vi "from string.vi"(8 "error in":errorcluster, 9 "data":string, 10 "version":string, 11 "Modbus Slave configuration in":refnum<class "Modbus Module configuration.lvclass">) -> (0 "error out":errorcluster, 3 "Modbus Slave configuration out":refnum<class "Modbus Module configuration.lvclass">)   [LabVIEW 2015, in "Modbus Module configuration.lvclass"]
doc: "Provides an interface for loading a module configuration from a file or other serialized data source. It is recommended that all children of this class store data in two sets--data required for its own initialization, and any data required for parent initialization--and that each implementation uses the <b>Call Parent Method</b> primitive to de-serialize parent information. As a result, it is expected that every module configuration class calls <b>component configuration.lvclass:From String.vi</b>.Platypus Framework 1.0.1.65\nNI Systems Engineering - National Instruments"
uses:
  Modbus Module configuration.lvclass
  module channel/Modbus Module Channel.lvclass
  modbus class.ctl
  Modbus Module configuration.lvclass/Modbus Module configuration.ctl
  <vilib>/NI/Tag Bus Module Framework/module configuration/TBM module configuration.lvclass
  <vilib>/NI/Configuration Framework/serializable configuration/NISE_CEF_serializable configuration.lvclass
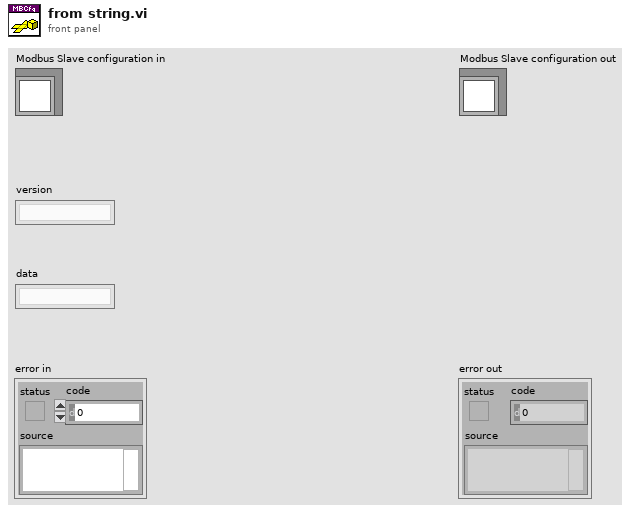
[diagram p1: front panel]
types:
  T1 = typedef "Modbus Module configuration.lvclass/modbus class.ctl" = enum16{"TCP master", "TCP slave", "serial master", "serial slave"}
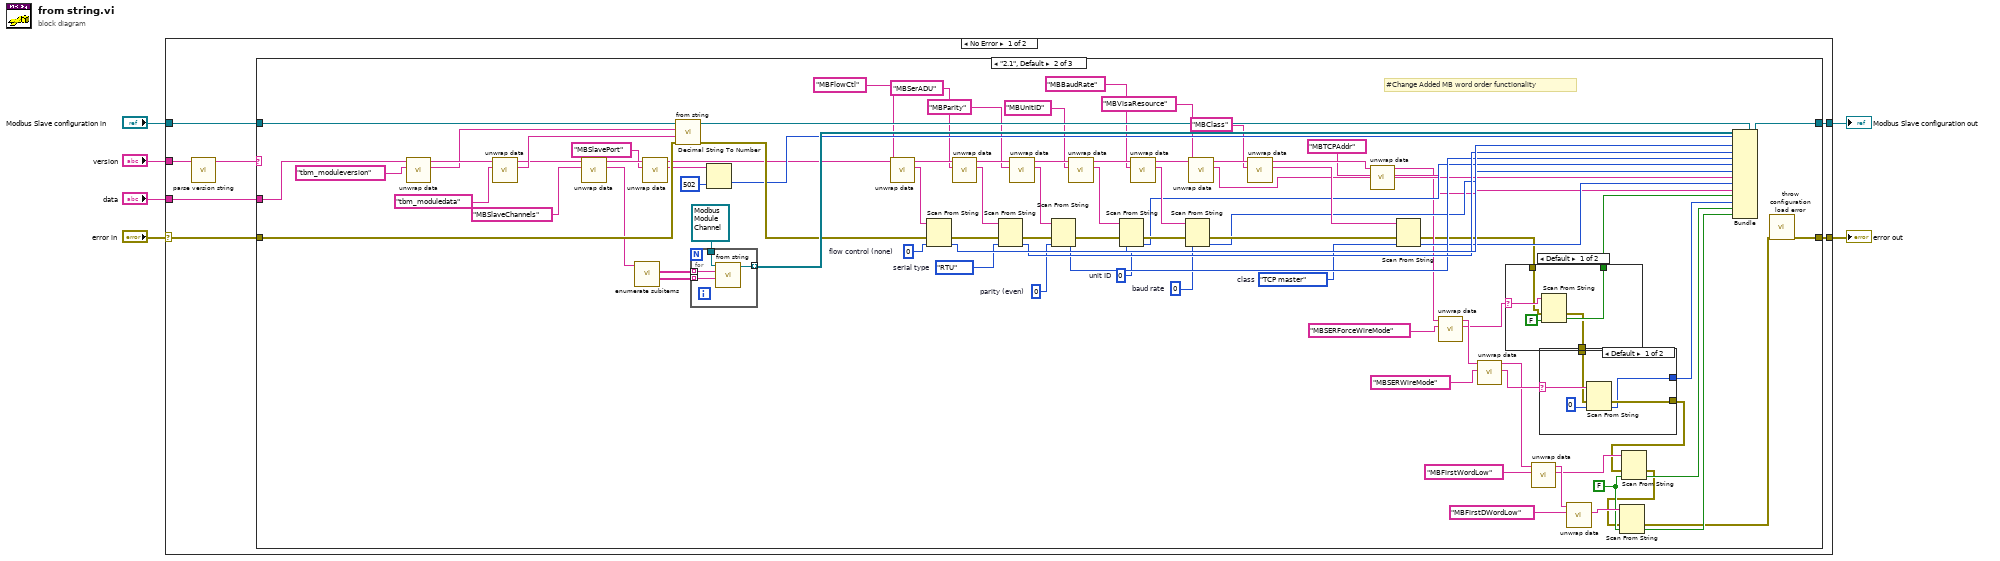
[diagram p0: block diagram]
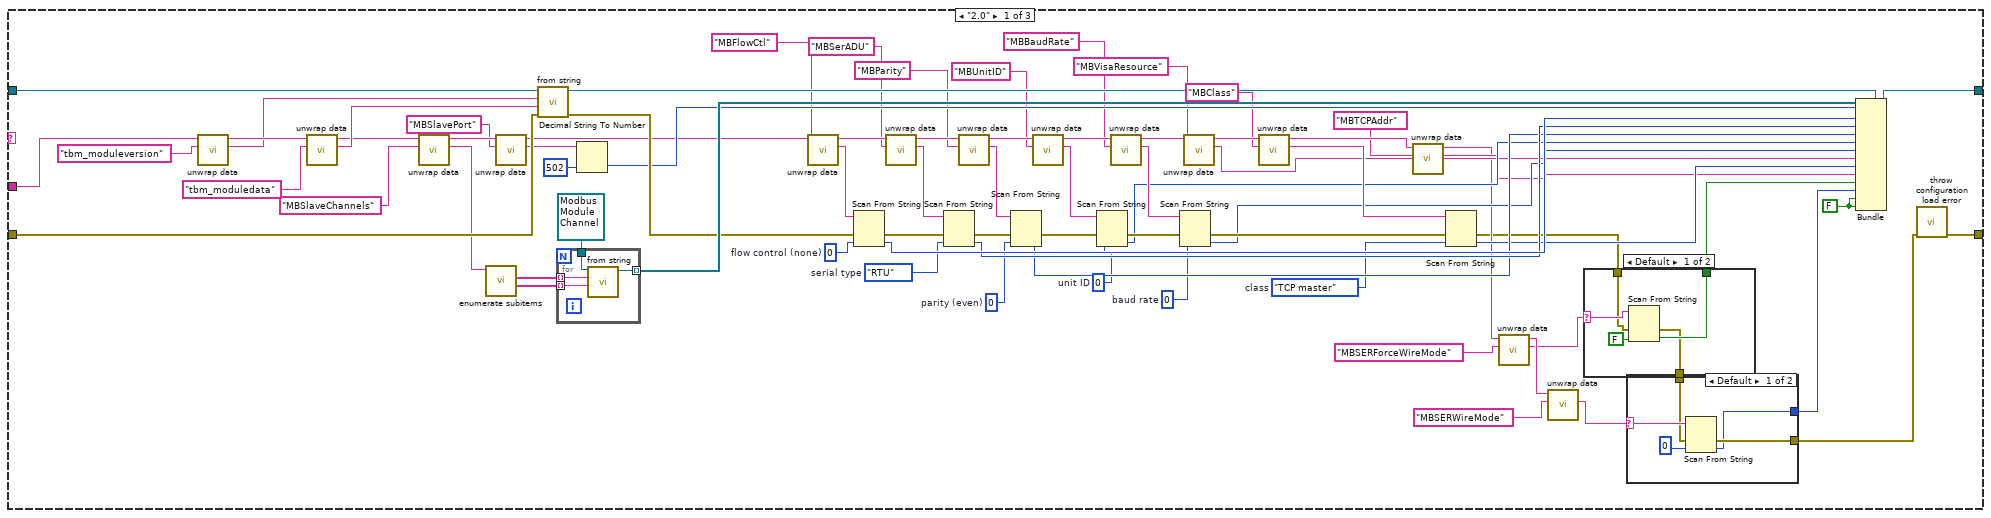
[diagram p2: hidden frame]
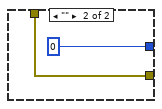
[diagram p3: hidden frame]
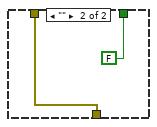
[diagram p4: hidden frame]
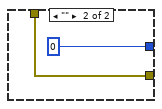
[diagram p5: hidden frame]
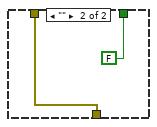
[diagram p6: hidden frame]
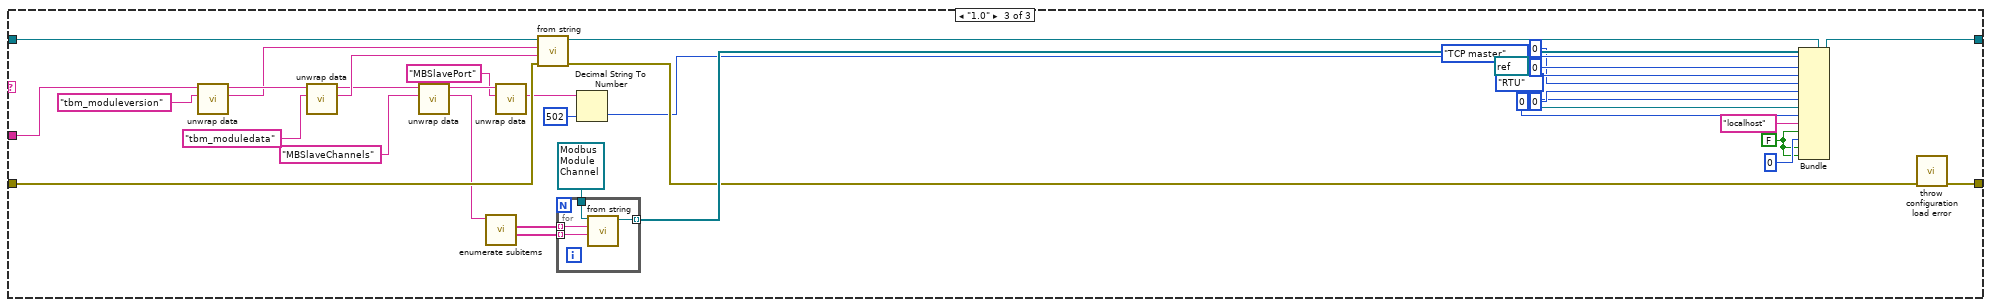
[diagram p7: hidden frame]
diagram:
  n1 = case shown="No Error" "error in" {
    selector: "error in" -> [w7 w253]
    tunnel: "data" -> [w13 _]
    tunnel: "Modbus Slave configuration in" -> [w12 w252]
    tunnel: [w11 w252] -> w5
    tunnel: [w10 w253] -> w4
    tunnel: "version" -> [w9 _]
    frame No Error {
      n2 = call <vilib>:"parse version string.vi"("full version"=w9) -> ("major.minor version"=w8:string)  [unwired: 7 in, 3 out]
      n3 = case shown="\"2.1\", Default" w8 {
        tunnel: w13 -> [w86 w191 w243]
        tunnel: w7 -> [w85 w190 w242]
        tunnel: w12 -> [w90 w195 w247]
        tunnel: [w80 w185 w237] -> w11
        tunnel: [w88 w193 w245] -> w10
        frame "2.0" {
          w14 = FALSE ("64-bit: first dword low")
          w29 = u32 0  # baud rate
          w30 = modbus_class."TCP master"  # class
          w31 = enum16{"RTU", "ASCII"}."RTU"  # serial type
          w32 = u16 0  # parity (even)
          w33 = u8 0  # unit ID
          w41 = u16 0  # flow control (none)
          n4 = call <vilib>:"unwrap data.vi"("identifier"="tbm_moduleversion" ("additional identifier"), "data to unwrap"=w86) -> ("unwrapped data"=w81:string, "remaining string"=w87:string)  [unwired: 8 in]
          n5 = call <vilib>:"unwrap data.vi"("identifier"="tbm_moduledata" ("additional identifier"), "data to unwrap"=w87) -> ("unwrapped data"=w83:string, "remaining string"=w79:string)  [unwired: 8 in]
          n6 = call <vilib>:"unwrap data.vi"("identifier"="MBSlaveChannels" ("additional identifier"), "data to unwrap"=w79) -> ("unwrapped data"=w77:string, "remaining string"=w72:string)  [unwired: 8 in]
          n7 = call <vilib>:"enumerate subitems.vi"("data to enumerate"=w77) -> ("associated data"=w75:string[], "discovered subitems"=w76:string[])  [unwired: 8 in, 1 out]
          n8 = call <vilib>:"unwrap data.vi"("identifier"="MBSlavePort" ("additional identifier"), "data to unwrap"=w72) -> ("unwrapped data"=w70:string, "remaining string"=w60:string)  [unwired: 8 in]
          n9 = call-parent "from string.vi"("error in"=w85, "data"=w83, "version"=w81, "module configuration in"=w90) -> ("error out"=w73:errorcluster, "module configuration out"=w89:refnum<class "Modbus Module configuration.lvclass">)  [unwired: 6 in]
          n10 = for {
            tunnel: w76 -> [w108] mode=indexing
            tunnel: w75 -> [w107] mode=indexing
            tunnel: [w106] -> w74 mode=indexing
            tunnel: refnum<class "Modbus Module Channel.lvclass"> refnum ("Modbus Module Channel.lvclass") -> [w105]
            n11 = call-dynamic "from string.vi"("channel data"=w107, "identifier"=w108, "channel in"=w105) -> ("channel out"=w106:refnum<class "Modbus Module Channel.lvclass">)  [unwired: 7 in, 1 out]
          }
          n12 = Decimal String To Number(string=w70, default (0L)=u16 502 ("default (0 I32)")) -> (number=w68:u16)  [unwired: 1 in, 1 out]
          n13 = call <vilib>:"unwrap data.vi"("identifier"="MBFlowCtl", "data to unwrap"=w60) -> ("unwrapped data"=w48:string, "remaining string"=w61:string)  [unwired: 8 in]
          n14 = Scan From String(input string=w48, error in=w73, default 1=w41) -> (error out=w51:errorcluster, output 1=w40:u16)  [unwired: 2 in, 2 out]
          n15 = call <vilib>:"unwrap data.vi"("identifier"="MBSerADU", "data to unwrap"=w61) -> ("unwrapped data"=w49:string, "remaining string"=w62:string)  [unwired: 8 in]
          n16 = Scan From String(input string=w49, error in=w51, default 1=w31) -> (error out=w50:errorcluster, output 1=w39:enum16{"RTU", "ASCII"})  [unwired: 2 in, 2 out]
          n17 = call <vilib>:"unwrap data.vi"("identifier"="MBParity", "data to unwrap"=w62) -> ("unwrapped data"=w47:string, "remaining string"=w63:string)  [unwired: 8 in]
          n18 = Scan From String(input string=w47, error in=w50, default 1=w32) -> (error out=w52:errorcluster, output 1=w38:u16)  [unwired: 2 in, 2 out]
          n19 = call <vilib>:"unwrap data.vi"("identifier"="MBUnitID", "data to unwrap"=w63) -> ("unwrapped data"=w45:string, "remaining string"=w64:string)  [unwired: 8 in]
          n20 = Scan From String(input string=w45, error in=w52, default 1=w33) -> (error out=w46:errorcluster, output 1=w37:u8)  [unwired: 2 in, 2 out]
          n21 = call <vilib>:"unwrap data.vi"("identifier"="MBBaudRate", "data to unwrap"=w64) -> ("unwrapped data"=w43:string, "remaining string"=w65:string)  [unwired: 8 in]
          n22 = Scan From String(input string=w43, error in=w46, default 1=w29) -> (error out=w44:errorcluster, output 1=w36:u32)  [unwired: 2 in, 2 out]
          n23 = call <vilib>:"unwrap data.vi"("identifier"="MBVisaResource", "data to unwrap"=w65) -> ("unwrapped data"=w34:string, "remaining string"=w66:string)  [unwired: 8 in]
          n24 = call <vilib>:"unwrap data.vi"("identifier"="MBClass", "data to unwrap"=w66) -> ("unwrapped data"=w42:string, "remaining string"=w28:string)  [unwired: 8 in]
          n25 = call <vilib>:"unwrap data.vi"("identifier"="MBTCPAddr", "data to unwrap"=w28) -> ("unwrapped data"=w26:string, "remaining string"=w25:string)  [unwired: 8 in]
          n26 = Scan From String(input string=w42, error in=w44, default 1=w30) -> (error out=w17:errorcluster, output 1=w35:T1)  [unwired: 2 in, 2 out]
          n27 = call <vilib>:"unwrap data.vi"("identifier"="MBSERForceWireMode", "data to unwrap"=w25) -> ("unwrapped data"=w21:string, "remaining string"=w24:string)  [unwired: 8 in]
          n28 = call <vilib>:"unwrap data.vi"("identifier"="MBSERWireMode", "data to unwrap"=w24) -> ("unwrapped data"=w20:string)  [unwired: 8 in, 1 out]
          n29 = case shown="Default" w21 {
            selector: w21 -> [w102 _]
            tunnel: [w100 FALSE] -> w18
            tunnel: w17 -> [w99 w103]
            tunnel: [w98 w103] -> w16
            frame Default {
              n30 = Scan From String(input string=w102, error in=w99, default 1=FALSE) -> (error out=w98:errorcluster, output 1=w100:bool)  [unwired: 2 in, 2 out]
            }
            frame "" {
            }
          }
          n31 = case shown="Default" w20 {
            selector: w20 -> [w95 _]
            tunnel: [w91 i16 0 ("Wire Mode")] -> w19
            tunnel: w16 -> [w93 w96]
            tunnel: [w92 w96] -> w15
            frame Default {
              n32 = Scan From String(input string=w95, error in=w93, default 1=i16 0 ("Wire Mode")) -> (error out=w92:errorcluster, output 1=w91:i16)  [unwired: 2 in, 2 out]
            }
            frame "" {
            }
          }
          n33 = Bundle(cluster=w89, w74, w68, w40, w39, w38, w37, w36, w34, w35, w26, w18, w19, w14, w14) -> (w80:refnum<class "Modbus Module configuration.lvclass">)
          n34 = call <vilib>:"throw configuration load error.vi"("error in"=w15) -> ("error out"=w88:errorcluster)  [unwired: 10 in]
        }
        frame "2.1", Default {
          w114 = FALSE ("64-bit: first dword low")
          w134 = u32 0  # baud rate
          w135 = modbus_class."TCP master"  # class
          w136 = enum16{"RTU", "ASCII"}."RTU"  # serial type
          w137 = u16 0  # parity (even)
          w138 = u8 0  # unit ID
          w146 = u16 0  # flow control (none)
          # "#Change Added MB word order functionality"
          n35 = call <vilib>:"unwrap data.vi"("identifier"="tbm_moduleversion" ("additional identifier"), "data to unwrap"=w191) -> ("unwrapped data"=w186:string, "remaining string"=w192:string)  [unwired: 8 in]
          n36 = call <vilib>:"unwrap data.vi"("identifier"="tbm_moduledata" ("additional identifier"), "data to unwrap"=w192) -> ("unwrapped data"=w188:string, "remaining string"=w184:string)  [unwired: 8 in]
          n37 = call <vilib>:"unwrap data.vi"("identifier"="MBSlaveChannels" ("additional identifier"), "data to unwrap"=w184) -> ("unwrapped data"=w182:string, "remaining string"=w177:string)  [unwired: 8 in]
          n38 = call <vilib>:"enumerate subitems.vi"("data to enumerate"=w182) -> ("associated data"=w180:string[], "discovered subitems"=w181:string[])  [unwired: 8 in, 1 out]
          n39 = call <vilib>:"unwrap data.vi"("identifier"="MBSlavePort" ("additional identifier"), "data to unwrap"=w177) -> ("unwrapped data"=w175:string, "remaining string"=w165:string)  [unwired: 8 in]
          n40 = call-parent "from string.vi"("error in"=w190, "data"=w188, "version"=w186, "module configuration in"=w195) -> ("error out"=w178:errorcluster, "module configuration out"=w194:refnum<class "Modbus Module configuration.lvclass">)  [unwired: 6 in]
          n41 = for {
            tunnel: w181 -> [w213] mode=indexing
            tunnel: w180 -> [w212] mode=indexing
            tunnel: [w211] -> w179 mode=indexing
            tunnel: refnum<class "Modbus Module Channel.lvclass"> refnum ("Modbus Module Channel.lvclass") -> [w210]
            n42 = call-dynamic "from string.vi"("channel data"=w212, "identifier"=w213, "channel in"=w210) -> ("channel out"=w211:refnum<class "Modbus Module Channel.lvclass">)  [unwired: 7 in, 1 out]
          }
          n43 = Decimal String To Number(string=w175, default (0L)=u16 502 ("default (0 I32)")) -> (number=w173:u16)  [unwired: 1 in, 1 out]
          n44 = call <vilib>:"unwrap data.vi"("identifier"="MBFlowCtl", "data to unwrap"=w165) -> ("unwrapped data"=w153:string, "remaining string"=w166:string)  [unwired: 8 in]
          n45 = Scan From String(input string=w153, error in=w178, default 1=w146) -> (error out=w156:errorcluster, output 1=w145:u16)  [unwired: 2 in, 2 out]
          n46 = call <vilib>:"unwrap data.vi"("identifier"="MBSerADU", "data to unwrap"=w166) -> ("unwrapped data"=w154:string, "remaining string"=w167:string)  [unwired: 8 in]
          n47 = Scan From String(input string=w154, error in=w156, default 1=w136) -> (error out=w155:errorcluster, output 1=w144:enum16{"RTU", "ASCII"})  [unwired: 2 in, 2 out]
          n48 = call <vilib>:"unwrap data.vi"("identifier"="MBParity", "data to unwrap"=w167) -> ("unwrapped data"=w152:string, "remaining string"=w168:string)  [unwired: 8 in]
          n49 = Scan From String(input string=w152, error in=w155, default 1=w137) -> (error out=w157:errorcluster, output 1=w143:u16)  [unwired: 2 in, 2 out]
          n50 = call <vilib>:"unwrap data.vi"("identifier"="MBUnitID", "data to unwrap"=w168) -> ("unwrapped data"=w150:string, "remaining string"=w169:string)  [unwired: 8 in]
          n51 = Scan From String(input string=w150, error in=w157, default 1=w138) -> (error out=w151:errorcluster, output 1=w142:u8)  [unwired: 2 in, 2 out]
          n52 = call <vilib>:"unwrap data.vi"("identifier"="MBBaudRate", "data to unwrap"=w169) -> ("unwrapped data"=w148:string, "remaining string"=w170:string)  [unwired: 8 in]
          n53 = Scan From String(input string=w148, error in=w151, default 1=w134) -> (error out=w149:errorcluster, output 1=w141:u32)  [unwired: 2 in, 2 out]
          n54 = call <vilib>:"unwrap data.vi"("identifier"="MBVisaResource", "data to unwrap"=w170) -> ("unwrapped data"=w139:string, "remaining string"=w171:string)  [unwired: 8 in]
          n55 = call <vilib>:"unwrap data.vi"("identifier"="MBClass", "data to unwrap"=w171) -> ("unwrapped data"=w147:string, "remaining string"=w133:string)  [unwired: 8 in]
          n56 = call <vilib>:"unwrap data.vi"("identifier"="MBTCPAddr", "data to unwrap"=w133) -> ("unwrapped data"=w131:string, "remaining string"=w130:string)  [unwired: 8 in]
          n57 = Scan From String(input string=w147, error in=w149, default 1=w135) -> (error out=w122:errorcluster, output 1=w140:T1)  [unwired: 2 in, 2 out]
          n58 = call <vilib>:"unwrap data.vi"("identifier"="MBSERForceWireMode", "data to unwrap"=w130) -> ("unwrapped data"=w126:string, "remaining string"=w129:string)  [unwired: 8 in]
          n59 = call <vilib>:"unwrap data.vi"("identifier"="MBSERWireMode", "data to unwrap"=w129) -> ("unwrapped data"=w125:string, "remaining string"=w118:string)  [unwired: 8 in]
          n60 = case shown="Default" w126 {
            selector: w126 -> [w207 _]
            tunnel: [w205 FALSE] -> w123
            tunnel: w122 -> [w204 w208]
            tunnel: [w203 w208] -> w121
            frame Default {
              n61 = Scan From String(input string=w207, error in=w204, default 1=FALSE) -> (error out=w203:errorcluster, output 1=w205:bool)  [unwired: 2 in, 2 out]
            }
            frame "" {
            }
          }
          n62 = call <vilib>:"unwrap data.vi"("identifier"="MBFirstWordLow", "data to unwrap"=w118) -> ("unwrapped data"=w116:string, "remaining string"=w117:string)  [unwired: 8 in]
          n63 = case shown="Default" w125 {
            selector: w125 -> [w200 _]
            tunnel: [w196 i16 0 ("Wire Mode")] -> w124
            tunnel: w121 -> [w198 w201]
            tunnel: [w197 w201] -> w111
            frame Default {
              n64 = Scan From String(input string=w200, error in=w198, default 1=i16 0 ("Wire Mode")) -> (error out=w197:errorcluster, output 1=w196:i16)  [unwired: 2 in, 2 out]
            }
            frame "" {
            }
          }
          n65 = call <vilib>:"unwrap data.vi"("identifier"="MBFirstDWordLow", "data to unwrap"=w117) -> ("unwrapped data"=w115:string)  [unwired: 8 in, 1 out]
          n66 = Scan From String(input string=w116, error in=w111, default 1=w114) -> (error out=w110:errorcluster, output 1=w113:bool)  [unwired: 2 in, 2 out]
          n67 = Scan From String(input string=w115, error in=w110, default 1=w114) -> (error out=w109:errorcluster, output 1=w112:bool)  [unwired: 2 in, 2 out]
          n68 = Bundle(cluster=w194, w179, w173, w145, w144, w143, w142, w141, w139, w140, w131, w123, w124, w113, w112) -> (w185:refnum<class "Modbus Module configuration.lvclass">)
          n69 = call <vilib>:"throw configuration load error.vi"("error in"=w109) -> ("error out"=w193:errorcluster)  [unwired: 10 in]
        }
        frame "1.0" {
          w214 = FALSE ("force wire mode")
          n70 = call <vilib>:"unwrap data.vi"("identifier"="tbm_moduleversion" ("additional identifier"), "data to unwrap"=w243) -> ("unwrapped data"=w238:string, "remaining string"=w244:string)  [unwired: 8 in]
          n71 = call <vilib>:"unwrap data.vi"("identifier"="tbm_moduledata" ("additional identifier"), "data to unwrap"=w244) -> ("unwrapped data"=w240:string, "remaining string"=w236:string)  [unwired: 8 in]
          n72 = call <vilib>:"unwrap data.vi"("identifier"="MBSlaveChannels" ("additional identifier"), "data to unwrap"=w236) -> ("unwrapped data"=w234:string, "remaining string"=w229:string)  [unwired: 8 in]
          n73 = call <vilib>:"enumerate subitems.vi"("data to enumerate"=w234) -> ("associated data"=w232:string[], "discovered subitems"=w233:string[])  [unwired: 8 in, 1 out]
          n74 = call <vilib>:"unwrap data.vi"("identifier"="MBSlavePort" ("additional identifier"), "data to unwrap"=w229) -> ("unwrapped data"=w227:string)  [unwired: 8 in, 1 out]
          n75 = call-parent "from string.vi"("error in"=w242, "data"=w240, "version"=w238, "module configuration in"=w247) -> ("error out"=w230:errorcluster, "module configuration out"=w246:refnum<class "Modbus Module configuration.lvclass">)  [unwired: 6 in]
          n76 = for {
            tunnel: w233 -> [w251] mode=indexing
            tunnel: w232 -> [w250] mode=indexing
            tunnel: [w249] -> w231 mode=indexing
            tunnel: refnum<class "Modbus Module Channel.lvclass"> refnum ("Modbus Module Channel.lvclass") -> [w248]
            n77 = call-dynamic "from string.vi"("channel data"=w250, "identifier"=w251, "channel in"=w248) -> ("channel out"=w249:refnum<class "Modbus Module Channel.lvclass">)  [unwired: 7 in, 1 out]
          }
          n78 = Decimal String To Number(string=w227, default (0L)=u16 502 ("default (0 I32)")) -> (number=w225:u16)  [unwired: 1 in, 1 out]
          n79 = Bundle(cluster=w246, w231, w225, u16 0 ("flow control (none)"), enum16{"RTU", "ASCII"}."RTU" ("serial type"), u16 0 ("parity (even)"), u8 0 ("unit ID"), u32 0 ("baud rate"), refnum<visa-resource-name> refnum ("VISA resource name"), modbus_class."TCP master" ("class"), "localhost" ("IP address"), w214, i16 0 ("Wire Mode"), w214, w214) -> (w237:refnum<class "Modbus Module configuration.lvclass">)
          n80 = call <vilib>:"throw configuration load error.vi"("error in"=w230) -> ("error out"=w245:errorcluster)  [unwired: 10 in]
        }
      }
    }
    frame Error {
    }
  }
  "error out" <- w4
  "Modbus Slave configuration out" <- w5
